vi "New RegReadExt Command.vi"(0 "RFFE RegReadExt Command in":refnum<class "RFFE RegReadExt Command.lvclass">, 1 "Alias":string, 5 "Slave Address":T2=12 format="%02x", 7 "Register Address":T1 format="%02x", 9 "Byte Count":i32=1, 11 "error in (no error)":errorcluster) -> (4 "RFFE RegReadExt Command out":refnum<class "RFFE RegReadExt Command.lvclass">, 15 "error out":errorcluster)   [LabVIEW 2018, in "MIPI RFFE API.lvlib" / "RFFE RegReadExt Command.lvclass"]
uses:
  RFFE RegReadExt Command.lvclass
  C:/Users/semoore/Projects/mipi-rffe-labview-oop/Extended Command/RFFE Extended Command.lvclass
  Slave Address.ctl
  Register Address.ctl
  Register Data.ctl
  RFFE RegReadExt Command.lvclass/RFFE RegReadExt Command.ctl
  Extended Command/RFFE Extended Command.lvclass
  MIPI RFFE API.lvlib
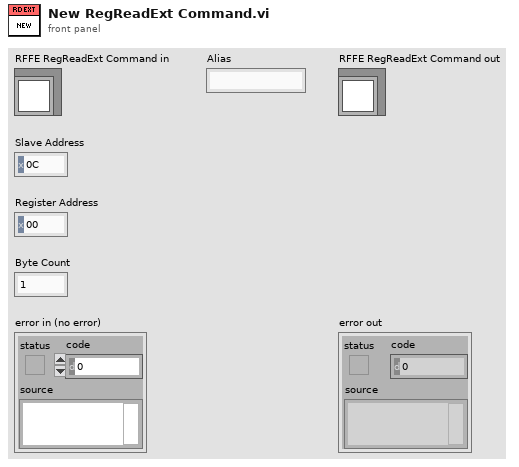
[diagram p1: front panel]
types:
  T1 = typedef "MIPI RFFE API.lvlib/Register Address.ctl" = u16
  T2 = typedef "MIPI RFFE API.lvlib/Slave Address.ctl" = u8
  T3 = typedef "MIPI RFFE API.lvlib/Register Data.ctl" = u8
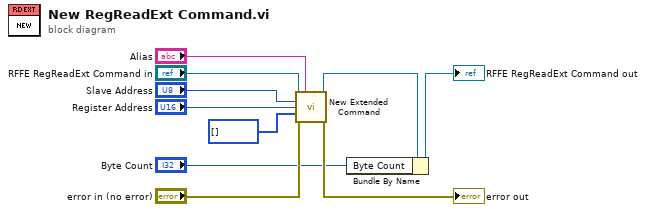
[diagram p0: block diagram]
diagram:
  n1 = call "New Extended Command.vi"("RFFE Extended Command in"="RFFE RegReadExt Command in", "Alias"="Alias", "Slave Address"="Slave Address", "Register Address"="Register Address", "Register Data"=T3[] [], "error in (no error)"="error in (no error)") -> ("RFFE Extended Command out"=w2:refnum<class "RFFE RegReadExt Command.lvclass">, "error out"=→"error out":errorcluster)  [unwired: 8 in]
  n2 = Bundle By Name(cluster=w2, "Byte Count"="Byte Count") -> (→"RFFE RegReadExt Command out":refnum<class "RFFE RegReadExt Command.lvclass">)
